vi "PIDAutoTune_SetTuningArguments.vi"(4 "Long Ave Time":i32=6, 5 "Controller Constant Type":T1(ring)=enum."Ziegler Nicols - Slow", 6 "Newest Avg Time":i32=1, 7 "Type of Controller":enum16{"P", "PI", "PID"}(ring)=enum."PI", 8 "Plant Tolerance":dbl=0.001, 9 "Tuning Tolerance":dbl=0.001, 10 "Kn":dbl=1.0, 11 "CO Offset":dbl=0.25) -> (3 "Configuration Parameters":T2={"Controller Constant Type"=enum."Ziegler Nicols - Normal", "Type of Controller"=enum."PI", "CO Offset"=0.25, "Kn"=1.0, "Tuning Tolerance"=0.001, "Plant Tolerance"=0.001, "Newest Avg Time "=1, "Long Ave Time"=6})   [LabVIEW 2019, in "Trajectory_Library.lvlib"]
doc: "Pack the individual PID AutoTune testing parameters into a data cluster for use with the PID AutoTune functions.\n\nInputs:\n -- Control Constant Type -- enum -- Desired PID performance. This guides the calculation of the tuning parameters after the system transfer function (plant) has been determined. This choice determines how agressive the PID is in controlling the system error. Choices are:\n - Ziegler Nicols - Fast\n - Ziegler Nicols - Normal\n - Ziegler Nicols - Slow\n - CHR Regulator - 0% Overshoot\n - CHR Regulator - 20% Overshoot\n - CHR Servo - 0% Overshoot\n - CHR Servo - 20% Overshoot\n\n-- Type of Controller -- enum -- Type of PID. Choices are:\n - P -- Proportional only\n - PI -- Proportional and Integral only\n - PID -- Full Proportional, Integral, Derivative.\n \n-- CO Offset -- double -- The amount to step the control output to perform the test\n-- Kn -- double -- Normaliztion constant. This is the same value that is used with the PID. This is normally Max CO / Max PV. If this isn't used, set the value to 1.0. (Optional. Default: 1.0)\n-- Tuning Tolerance -- double -- Value used to determine if the tuning is complete. (Optional. Default 0.001)\n-- Plant Tolerance -- double -- Value used to determine if the tuning process is complete. (Optional. Default: 0.001)\n-- Newest Avg Time -- double -- Time in seconds to average most recent calculated tuning constants. (Optional. Default: 1.0 )\n-- Long Avg Time -- double -- Time in seconds to average tuning constants to determine if the values are still changing. (Optional. Default 6.0 )\n\nOutputs:\n -- Configuration Parameters -- cluster -- This contains the parameters defining the conditions of the test. Use the Pack routine to create this data cluster."
uses:
  Trajectory_Library.lvlib
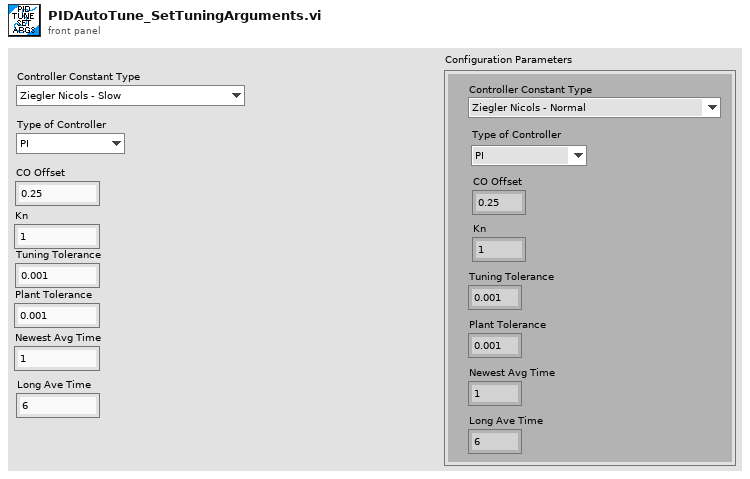
[diagram p1: front panel]
types:
  T1 = enum16{"Ziegler Nicols - Fast", "Ziegler Nicols - Normal", "Ziegler Nicols - Slow", "CHR regulator - 0% overshoot", "CHR regulator - 20% overshoot", "CHR servo - 0 % overshoot", "CHR servo - 20% overshoot"}
  T2 = cluster{"Controller Constant Type":enum16{"Ziegler Nicols - Fast", "Ziegler Nicols - Normal", "Ziegler Nicols - Slow", "CHR regulator - 0% overshoot", "CHR regulator - 20% overshoot", "CHR servo - 0 % overshoot", "CHR servo - 20% overshoot"}, "Type of Controller":enum16{"P", "PI", "PID"}, "CO Offset":dbl, "Kn":dbl, "Tuning Tolerance":dbl, "Plant Tolerance":dbl, "Newest Avg Time ":i32, "Long Ave Time":i32}
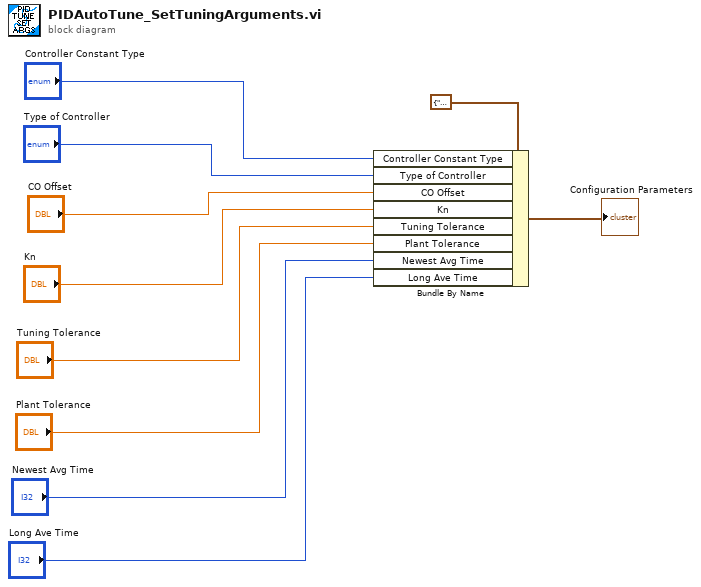
[diagram p0: block diagram]
diagram:
  n1 = Bundle By Name(cluster=T2 {"Controller Constant Type"=enum."Ziegler Nicols - Normal", "Type of Controller"=enum."PI", "CO Offset"=0.25, "Kn"=1.0, "Tuning Tolerance"=0.001, "Plant Tolerance"=0.001, "Newest Avg Time "=1, "Long Ave Time"=6} ("Tuning Parameters 2"), "Controller Constant Type"="Controller Constant Type", "Type of Controller"="Type of Controller", "CO Offset"="CO Offset", "Kn"="Kn", "Tuning Tolerance"="Tuning Tolerance", "Plant Tolerance"="Plant Tolerance", "Newest Avg Time"="Newest Avg Time", "Long Ave Time"="Long Ave Time") -> (→"Configuration Parameters":T2)
